vi "Vacum Valve Control.vi"(8 "error in":errorcluster, 11 "HTS Results in":refnum<class "HTS Results.lvclass">) -> (0 "error out":errorcluster, 1 "Valve Pos":dbl, 2 "Vavum Valve CMD":string="s", 3 "HTS Results out":refnum<class "HTS Results.lvclass">)   [LabVIEW 2019, in "Results.lvlib" / "HTS Results.lvclass"]
uses:
  HTS Results.lvclass
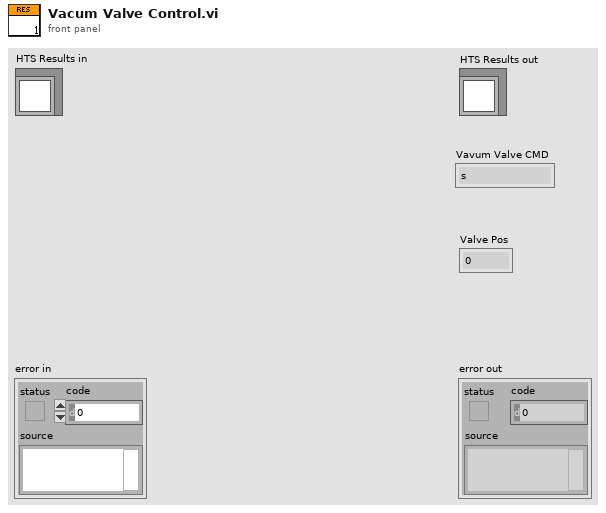
[diagram p1: front panel]
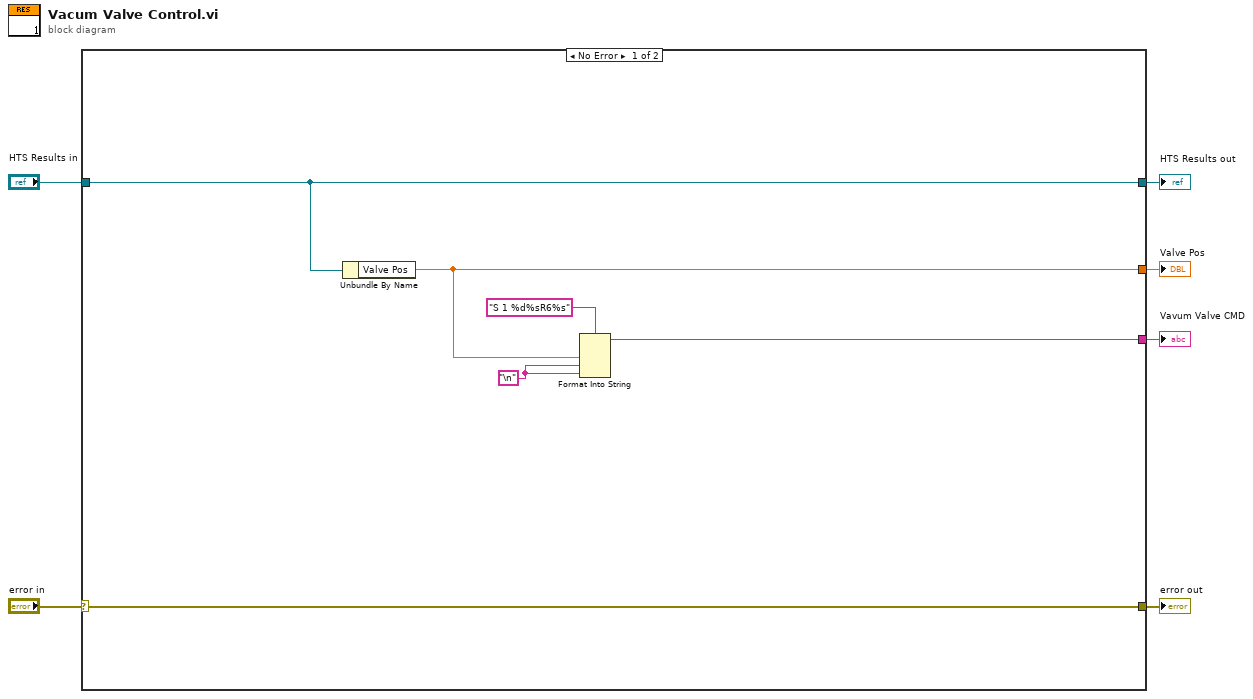
[diagram p0: block diagram]
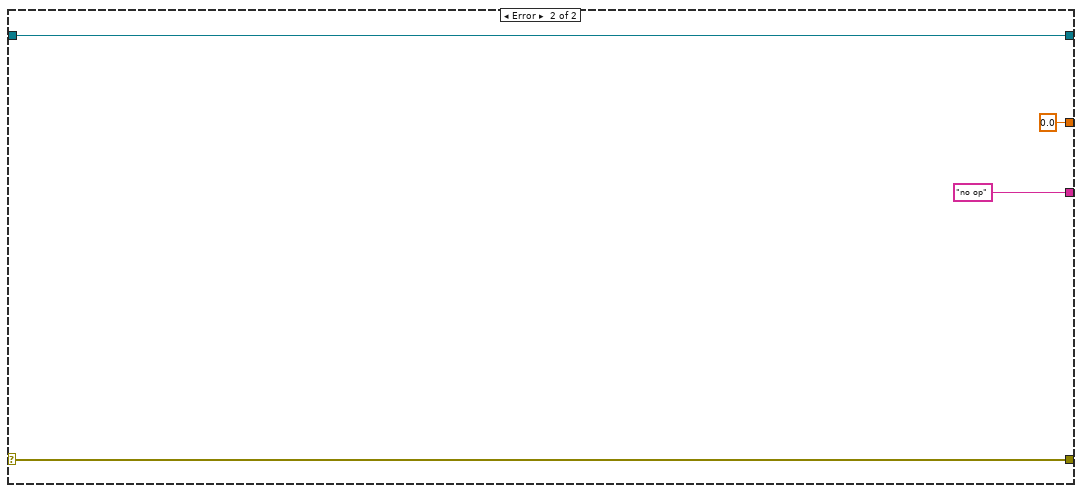
[diagram p2: hidden frame]
diagram:
  n1 = case shown="No Error" "error in" {
    selector: "error in" -> [w7 w16]
    tunnel: [w7 w16] -> w5
    tunnel: "HTS Results in" -> [w12 w15]
    tunnel: [w12 w15] -> w3
    tunnel: [w11 "no op"] -> w2
    tunnel: [w10 0.0 ("Valve Pos")] -> w1
    frame No Error {
      w8 = "\n"
      n2 = Unbundle By Name(w12) -> ("Valve Pos"=w10:dbl)
      n3 = Format Into String(format string="S 1 %d%sR6%s", w10, w8, w8) -> (resulting string=w11:string)  [unwired: 2 in, 1 out]
    }
    frame Error {
    }
  }
  "error out" <- w5
  "HTS Results out" <- w3
  "Vavum Valve CMD" <- w2
  "Valve Pos" <- w1
